vi "Wait for Turn Table Movement Complete.vi"(8 "error in (no error)":errorcluster, 11 "CO3000 in":refnum<class "CO3000.lvclass">) -> (0 "error out":errorcluster, 3 "CO3000 out":refnum<class "CO3000.lvclass">)   [LabVIEW 2023, in "Turn Table and Mast.lvlib" / "CO3000.lvclass"]
uses:
  CO3000.lvclass
  CO3000.lvclass/CO3000.ctl
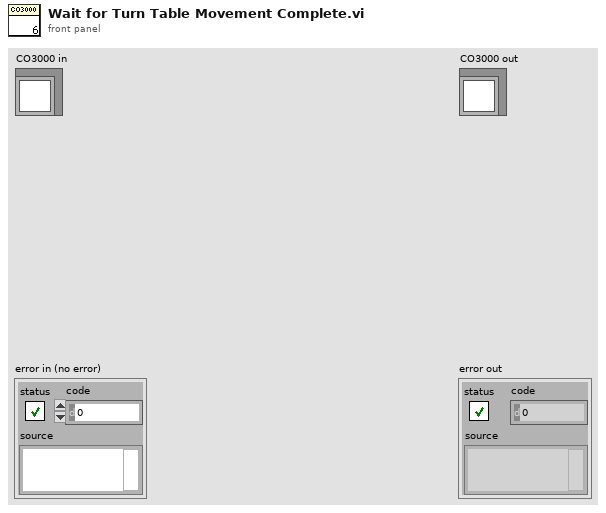
[diagram p1: front panel]
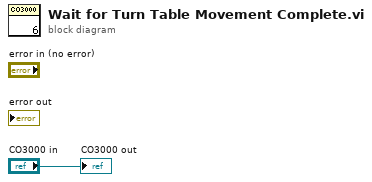
[diagram p0: block diagram]
diagram:
  "CO3000 out" <- "CO3000 in"
